vi "LTE Change RB Status.vi"(8 "error in (no error)":errorcluster caption="에러 입력(에러 없음)", 10 "RB Offset":i32, 11 "Instrument Manager 입력":refnum<class "Instrument Manager.lvclass">) -> (0 "error out":errorcluster caption="에러 출력", 3 "Instrument Manager 출력":refnum<class "Instrument Manager.lvclass">)   [LabVIEW 2023, in "Instrument Manager.lvclass"]
uses:
  Instrument Manager.lvclass
  Instrument Manager.lvclass/Instrument Manager.ctl
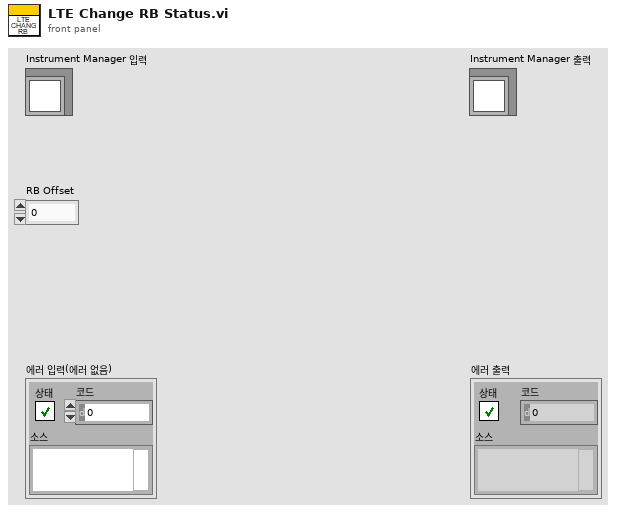
[diagram p1: front panel]
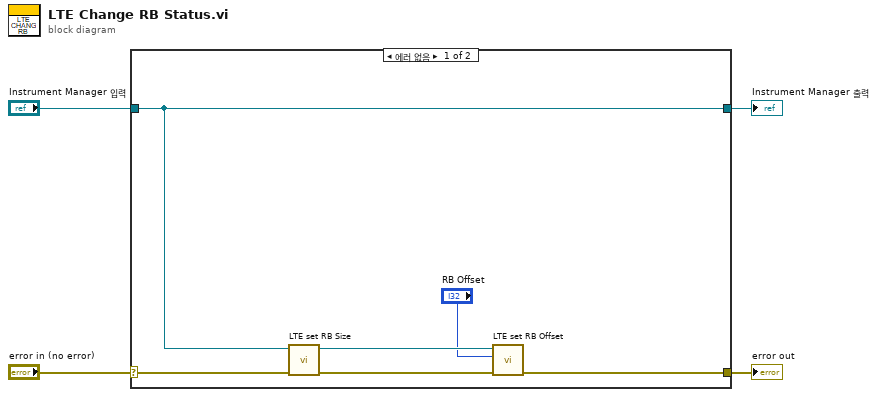
[diagram p0: block diagram]
diagram:
  n1 = case shown="에러 없음" "error in (no error)" {
    selector: "error in (no error)" -> [w10 w12]
    tunnel: [w8 w12] -> w3
    tunnel: [w7 w11] -> w1
    tunnel: "Instrument Manager 입력" -> [w7 w11]
    frame No Error {
      n2 = call "LTE set RB Size.vi"("error in (no error)"=w10, "Instrument Manager 입력"=w7) -> ("error out"=w9:errorcluster, "Instrument Manager 출력"=w6:refnum<class "Instrument Manager.lvclass">)  [unwired: 8 in]
      n3 = call "LTE set RB Offset.vi"("error in (no error)"=w9, "RB Offset"="RB Offset", "Instrument Manager 입력"=w6) -> ("error out"=w8:errorcluster)  [unwired: 7 in, 1 out]
    }
    frame Error {
    }
  }
  "error out" <- w3
  "Instrument Manager 출력" <- w1
